vi "Main.vi"(11 "Module Admin":refnum<class "Delacor_lib_QMH_Module Admin.lvclass">) -> ()   [LabVIEW 2026, in "My Singleton Module.lvlib"]
doc: "This template is based off of the Queued Message Handler design pattern and the Queued Message Handler project template that ships with LabVIEW.\n\nThe main difference is that the queue is private to this module and communication between modules is performed via Broadcast and Request events.\n\nRequest events are wrapped in public API methods and are handled in the Event Handling Loop (EHL) of this VI. Any module can register for Broadcast events sent by this module. The EHL generates messages based on user interface actions.\n\nThe Message Handling Loop (MHL) processes messages generated by the EHL, or by other messages. The messages are string values, so new messages can be added easily to the Message Cases case structure in the MHL. Each message cluster can also provide an optional value for Message Data, which is a variant that can be converted to whatever message-specific data is required.\n_____\nBased on DQMH Dev Tools: Project Template 7.1.2.1547."
uses:
  My Singleton Module.lvlib
  <vilib>/Delacor/Delacor QMH/Libraries/Module Admin_class/Delacor_lib_QMH_Module Admin.lvclass
  Module Data--cluster.ctl
  Do Something Argument--cluster.ctl
  <vilib>/Delacor/Delacor QMH/Libraries/Message Queue_class/Delacor_lib_QMH_Message Queue.lvclass/Delacor_lib_QMH_Message Queue.ctl
  Do Something Else Argument--cluster.ctl
  Do Something Else and Wait for Reply Argument--cluster.ctl
  Do Something Else and Wait (Reply Payload)--cluster.ctl
  Stop Argument--cluster.ctl
  <vilib>/Delacor/Delacor QMH/Libraries/Module Admin_class/Delacor_lib_QMH_Module Admin.lvclass/Delacor_lib_QMH_Module Admin.ctl
  Suma 2 Numeros Argument--cluster.ctl
  Suma 2 Numeros (Reply Payload)--cluster.ctl
  Crear Canales DAQ Argument--cluster.ctl
  Start Acquisition Argument--cluster.ctl
  Acquire Argument--cluster.ctl
  Acquire (Reply Payload)--cluster.ctl
  Stop Acquiring Argument--cluster.ctl
  <vilib>/Utility/miscctls.llb/LVPointTypeDef.ctl
  <vilib>/Delacor/Delacor QMH/Libraries/Message Queue_class/Delacor_lib_QMH_Enqueue Message (Single).vi
  <vilib>/Delacor/Delacor QMH/Libraries/Module Admin_class/Delacor_lib_QMH_Get External Launch.vi
  <vilib>/DAQmx/read.llb/DAQmx Read (Analog 1D Wfm NChan NSamp).vi
  <vilib>/DAQmx/miscellaneous.llb/DAQmx Fill In Error Info.vi
  <vilib>/Delacor/Delacor QMH/Libraries/Message Queue_class/Delacor_lib_QMH_Message Queue.lvclass
  DAQ/DAQ.lvlib
panel:
  out "error out":errorcluster
  out "X":dbl
  out "Status":string
  in  "Simulate MHL Error":bool
  in  "Simulate EHL Error":bool
  in  "Do Something Else <Replace Me>":bool
  in  "Do Something <Replace Me>":bool
  # "These controls have associated \"Value Changed\" events configured in the Event Structure on the diagram.\n\nReplace them (and reconfigure the Event Structure) with the controls you need for your application. \n\nOther processes communicate with this Module via its Public API (wrappers for its Request Events).\n\nThis Module communicates with other processes via its Broadcast Events.\nAny process that wants to receive these messages can register for this module's Broadcast events."
  # "This template is for the DQMH framework. See the block diagram for more information on how to use this template."
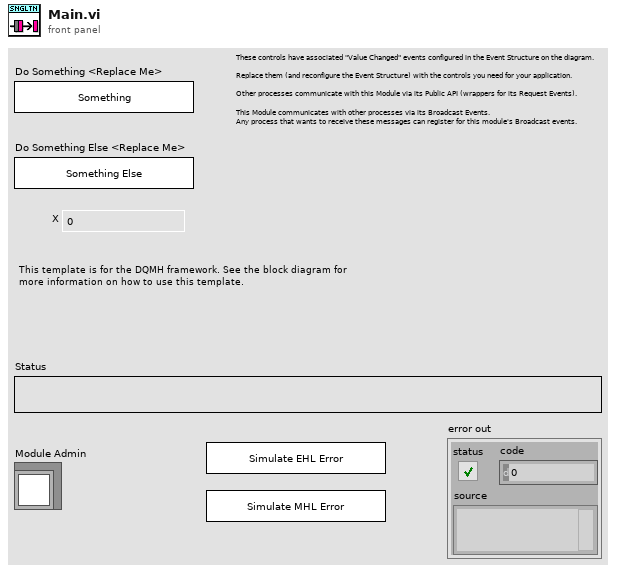
[diagram p1: front panel]
types:
  T1 = typedef "My Singleton Module.lvlib/Request Events--cluster.ctl" = cluster{"Stop Module":refnum<user-event>, "Do Something":refnum<user-event>, "Do Something Else":refnum<user-event>, "Do Something Else and Wait for Reply":refnum<user-event>, "Show Panel":refnum<user-event>, "Hide Panel":refnum<user-event>, "Get Module Execution Status":refnum<user-event>, "Show Diagram":refnum<user-event>, "Suma 2 Numeros":refnum<user-event>, "Crear Canales DAQ":refnum<user-event>, "Start Acquisition":refnum<user-event>, "Acquire":refnum<user-event>, "Stop Acquiring":refnum<user-event>}
  T2 = typedef "My Singleton Module.lvlib/Module Data--cluster.ctl" = cluster{"Status":string, "task out":refnum<k21>}
  T3 = typedef "My Singleton Module.lvlib/Do Something Argument--cluster.ctl" = cluster{"Do Something Msg":string}
  T4 = typedef "My Singleton Module.lvlib/Do Something Else Argument--cluster.ctl" = cluster{"Do Something Else Msg":string, "X":dbl}
  T5 = typedef "My Singleton Module.lvlib/Do Something Else and Wait for Reply Argument--cluster.ctl" = cluster{"Do Something Else Msg":string, "X":dbl, "Wait Notifier":refnum<notifier>, "wait for reply":bool}
  T6 = enum32{"invalid lock state", "Not Locked", "Locked (No Password)", "Password-protected"}
  T7 = typedef "My Singleton Module.lvlib/Stop Argument--cluster.ctl" = cluster{"Origin":string, "Exit via Stop Module Req?":bool, "Wait for Module to stop?":bool}
  T8 = typedef "My Singleton Module.lvlib/Suma 2 Numeros Argument--cluster.ctl" = cluster{"A":dbl, "B":dbl, "Wait Notifier":refnum<notifier>, "wait for reply":bool}
  T9 = typedef "My Singleton Module.lvlib/Crear Canales DAQ Argument--cluster.ctl" = cluster{"Boolean":bool}
  T10 = typedef "My Singleton Module.lvlib/Start Acquisition Argument--cluster.ctl" = cluster{"Boolean":bool}
  T11 = typedef "My Singleton Module.lvlib/Acquire Argument--cluster.ctl" = cluster{"Wait Notifier":refnum<notifier>, "wait for reply":bool}
  T12 = typedef "My Singleton Module.lvlib/Stop Acquiring Argument--cluster.ctl" = cluster{"Boolean":bool}
  T13 = typedef "LVPointTypeDef.ctl" = cluster{"Horizontal":i16, "Vertical":i16}
  T14 = enum32{"Invalid", "Standard", "Closed", "Hidden", "Minimized", "Maximized"}
  T15 = typedef "My Singleton Module.lvlib/Do Something Else and Wait (Reply Payload)--cluster.ctl" = cluster{"Value":dbl, "error":errorcluster}
  T16 = typedef "My Singleton Module.lvlib/Suma 2 Numeros (Reply Payload)--cluster.ctl" = cluster{"A+B":dbl, "error":errorcluster}
  T17 = typedef "My Singleton Module.lvlib/Acquire (Reply Payload)--cluster.ctl" = cluster{"data":waveform(dbl)[], "error":errorcluster}
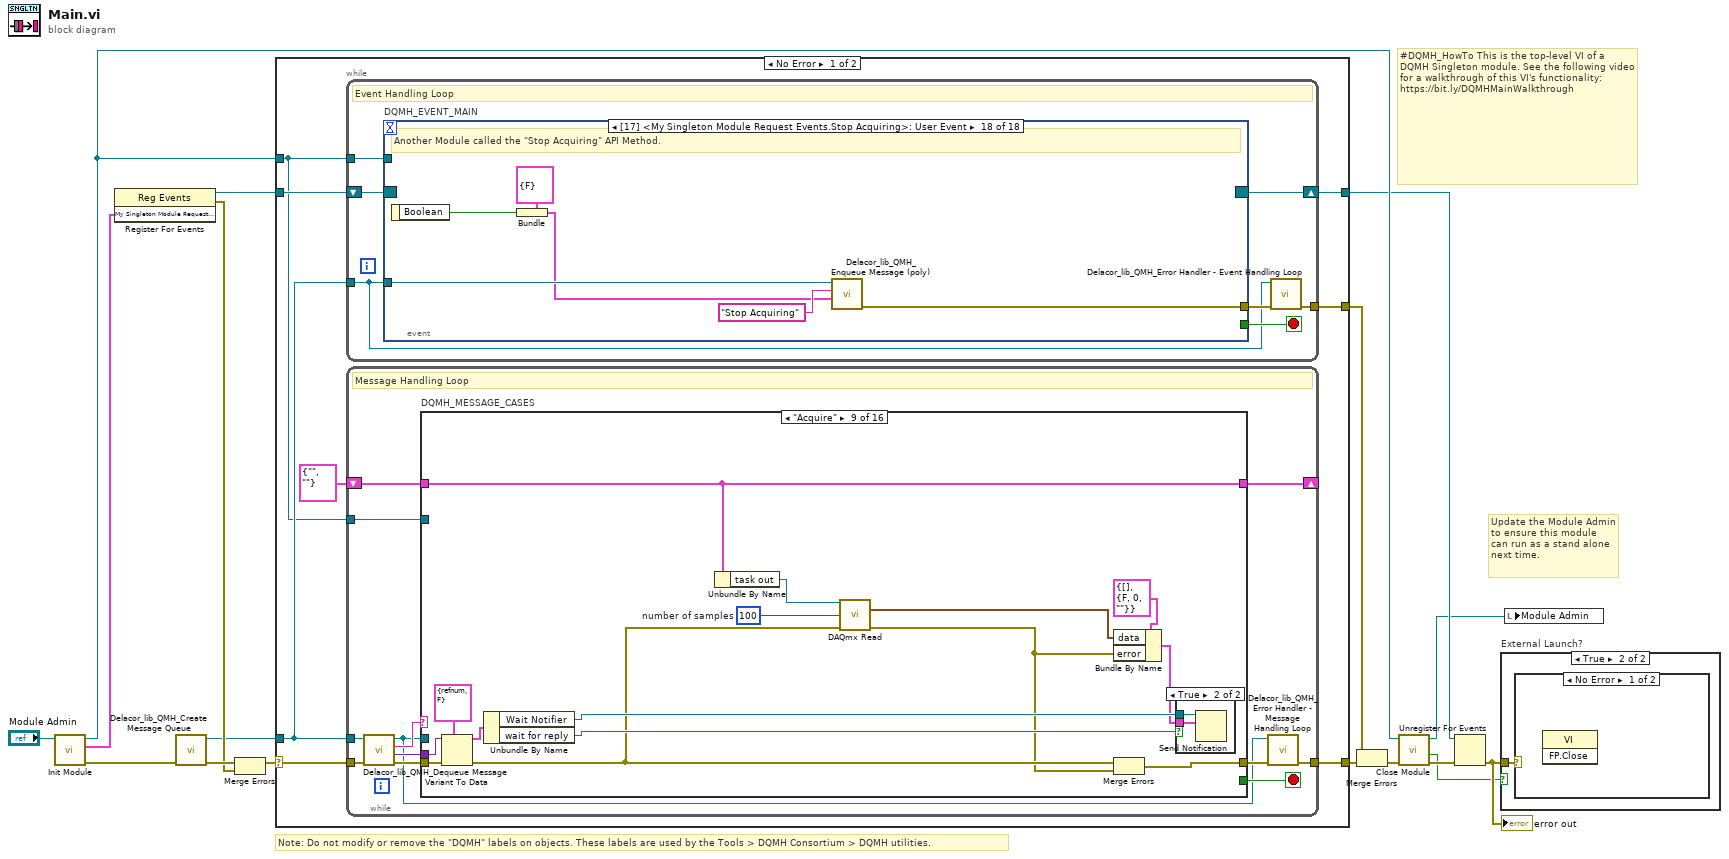
[diagram p0: block diagram]
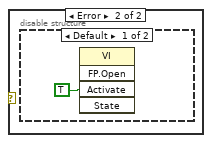
[diagram p3: hidden frame]
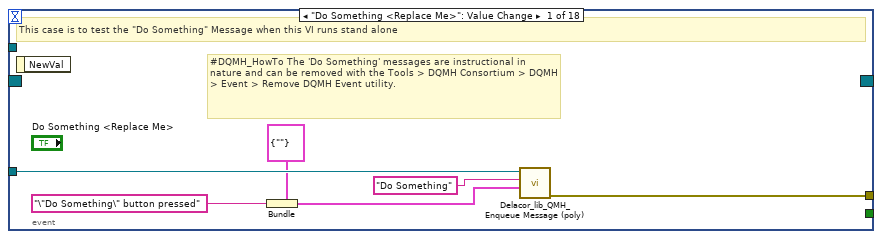
[diagram p5: hidden frame]
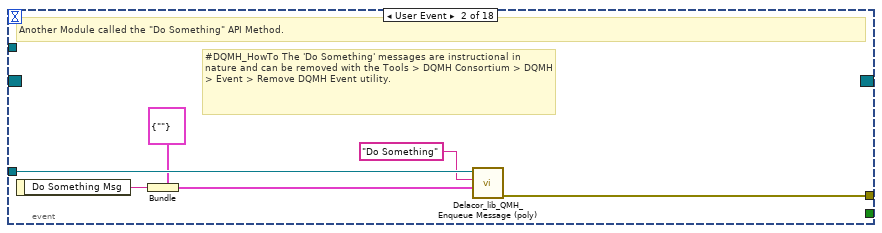
[diagram p6: hidden frame]
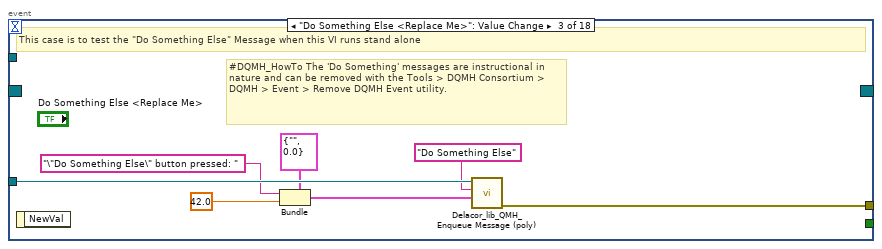
[diagram p7: hidden frame]
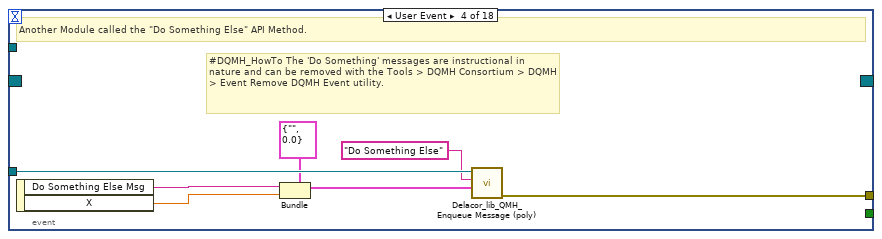
[diagram p8: hidden frame]
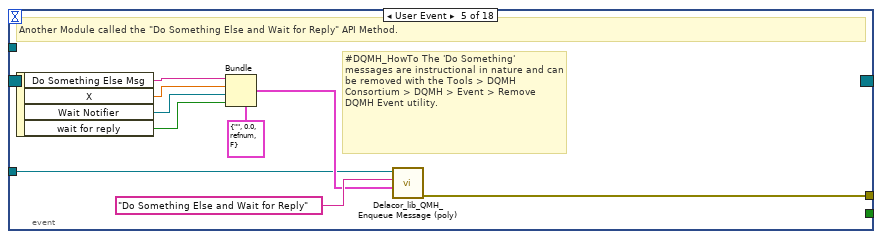
[diagram p9: hidden frame]
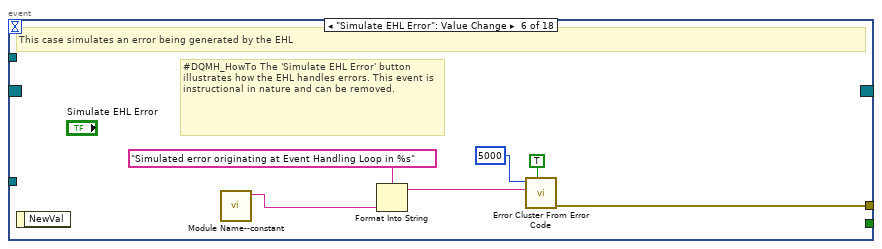
[diagram p10: hidden frame]
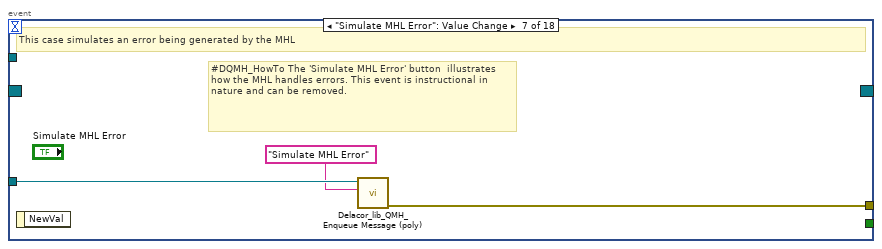
[diagram p11: hidden frame]
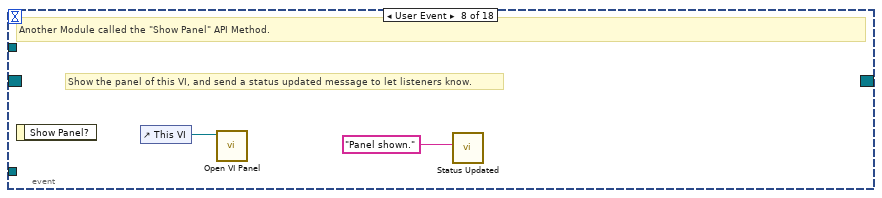
[diagram p12: hidden frame]
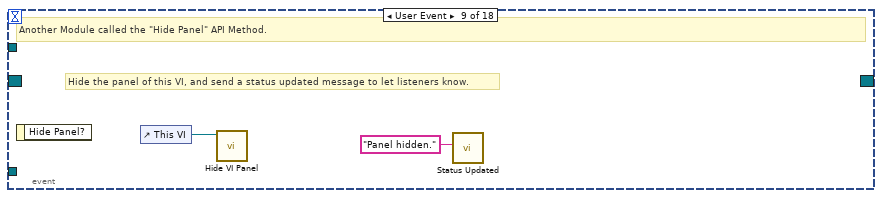
[diagram p13: hidden frame]
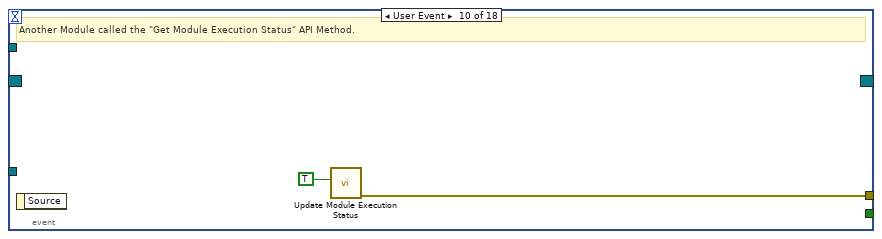
[diagram p14: hidden frame]
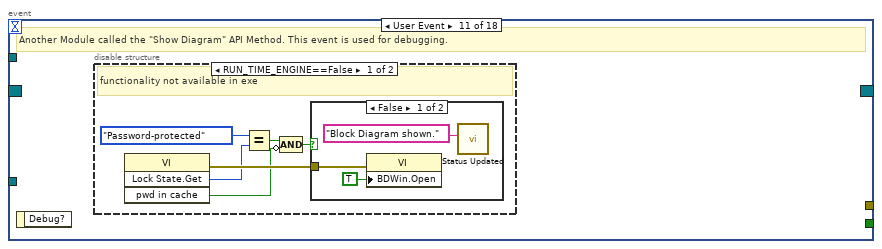
[diagram p15: hidden frame]
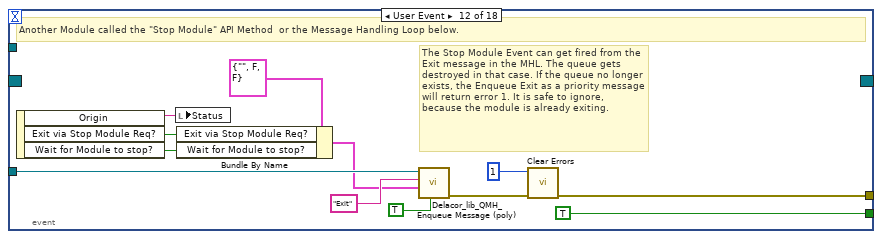
[diagram p18: hidden frame]
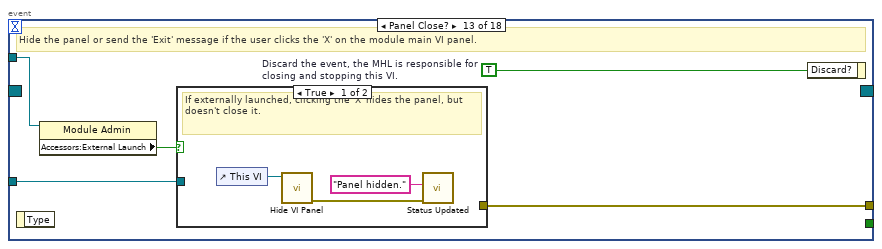
[diagram p19: hidden frame]
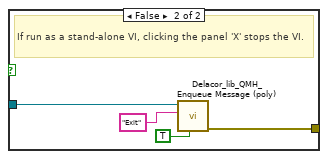
[diagram p20: hidden frame]
diagram:
  # "#DQMH_HowTo This is the top-level VI of a DQMH Singleton module. See the following video for a walkthrough of this VI's functionality: https://bit.ly/DQMHMainWalkthrough"
  # "Note: Do not modify or remove the \"DQMH\" labels on objects. These labels are used by the Tools > DQMH Consortium > DQMH utilities."
  # "Update the Module Admin to ensure this module can run as a stand alone next time."
  n1 = call "Init Module.vi"("Singleton Module Admin in"="Module Admin") -> ("error out"=w16:errorcluster, "My Singleton Module Request Events"=w5:T1, "Singleton Module Admin out"=w8:refnum<class "Delacor_lib_QMH_Module Admin.lvclass">)  [unwired: 8 in]
  n2 = register-events ("DQMH_REG_EVENTS")(w5) -> (reference out=w6:refnum<event-registration>, error out=w9:errorcluster)  [unwired: 2 in]
  n3 = call <vilib>:"Delacor_lib_QMH_Create Message Queue.vi"("error in"=w16) -> ("error out"=w11:errorcluster, "Message Queue"=w4:refnum<class "Delacor_lib_QMH_Message Queue.lvclass">)  [unwired: 9 in]
  n4 = Merge Errors(w11, w9) -> (w10:errorcluster)
  n5 = case shown="No Error" w10 {
    selector: w10 -> [w23 w357]
    tunnel: [w25 w356] -> w17
    tunnel: [w22 w355] -> w7
    tunnel: w6 -> [w20 w355]
    tunnel: w4 -> [w19 w350]
    tunnel: [w24 _] -> w14
    tunnel: w8 -> [w18 w351]
    frame No Error {
      n6 = while {
        tunnel: w19 -> [w26]
        shift-right: [w29] -> w22
        shift-left: w20 -> [w30]
        tunnel: [w31] -> w24
        tunnel: w18 -> [w27]
        stop <- w28 stop-if-true
        # "Event Handling Loop"
        n7 = event "DQMH_EVENT_MAIN" shown="[17] <My Singleton Module Request Events.Stop Acquiring>: User Event" {
          selector: w30 -> [_ _ _ _ _ _ _ _ _ _ _ _ _ _ _ _ _ _]
          dyn-events: [_ _ _ _ _ _ _ _ _ _ _ _ _ _ _ _ _ _] -> w29
          timeout: _ -> [_ _ _ _ _ _ _ _ _ _ _ _ _ _ _ _ _ _]
          tunnel: [_ _ _ _ _ _ _ _ _ _ _ TRUE ("Discard?") _ _ _ _ _ _] -> w28
          tunnel: w26 -> [w37 w43 w50 w57 w60 _ w75 _ _ _ _ w99 w106 w124 w130 w136 w143 w149]
          tunnel: [w38 w44 w51 w58 w67 w73 w76 _ _ w82 _ w102 w108 w116 w125 w133 w137 w144] -> w32
          tunnel: w27 -> [_ _ _ _ _ _ _ _ _ _ _ _ w105 _ _ _ _ _]
          event "Do Something <Replace Me>": Value Change {
            # "#DQMH_HowTo The 'Do Something' messages are instructional in nature and can be removed with the Tools > DQMH Consortium > DQMH > Event > Remove DQMH Event utility."
            # "This case is to test the \"Do Something\" Message when this VI runs stand alone"
            n8 = event-data() -> ()  [unwired: 1 in, 1 out]
            n9 = Bundle(cluster=T3 {"Do Something Msg"=""} ("Do Something Argument"), "Do Something Msg"="\"Do Something\" button pressed" ("\"Do Something\" button pressed")) -> (w33:T3)
            n10 = call-poly <vilib>:"Delacor_lib_QMH_Enqueue Message (poly).vi"("Message Data"=w33, "Message"="Do Something", "Message Queue in"=w37) -> ("error out"=w38:errorcluster)  [unwired: 7 in, 1 out]
          }
          event User Event {
            # "#DQMH_HowTo The 'Do Something' messages are instructional in nature and can be removed with the Tools > DQMH Consortium > DQMH > Event > Remove DQMH Event utility."
            # "Another Module called the \"Do Something\" API Method."
            n11 = event-data() -> ("Do Something Msg"=w40:string)  [unwired: 1 in]
            n12 = Bundle(cluster=T3 {"Do Something Msg"=""} ("Do Something Argument"), "Do Something Msg"=w40) -> (w39:T3)
            n13 = call-poly <vilib>:"Delacor_lib_QMH_Enqueue Message (poly).vi"("Message Data"=w39, "Message"="Do Something", "Message Queue in"=w43) -> ("error out"=w44:errorcluster)  [unwired: 7 in, 1 out]
          }
          event "Do Something Else <Replace Me>": Value Change {
            # "#DQMH_HowTo The 'Do Something' messages are instructional in nature and can be removed with the Tools > DQMH Consortium > DQMH > Event > Remove DQMH Event utility."
            # "This case is to test the \"Do Something Else\" Message when this VI runs stand alone"
            n14 = event-data() -> ()  [unwired: 1 in, 1 out]
            n15 = Bundle(cluster=T4 {"Do Something Else Msg"="", "X"=0.0} ("Do Something Else Argument"), "Do Something Else Msg"="\"Do Something Else\" button pressed: " ("\"Do Something Else\" button pressed"), "X"=42.0) -> (w47:T4)
            n16 = call-poly <vilib>:"Delacor_lib_QMH_Enqueue Message (poly).vi"("Message Data"=w47, "Message"="Do Something Else", "Message Queue in"=w50) -> ("error out"=w51:errorcluster)  [unwired: 7 in, 1 out]
          }
          event User Event {
            # "#DQMH_HowTo The 'Do Something' messages are instructional in nature and can be removed with the Tools > DQMH Consortium > DQMH > Event Remove DQMH Event utility."
            # "Another Module called the \"Do Something Else\" API Method."
            n17 = event-data() -> ("Do Something Else Msg"=w53:string, "X"=w52:dbl)  [unwired: 1 in]
            n18 = Bundle(cluster=T4 {"Do Something Else Msg"="", "X"=0.0} ("Do Something Else Argument"), "Do Something Else Msg"=w53, "X"=w52) -> (w54:T4)
            n19 = call-poly <vilib>:"Delacor_lib_QMH_Enqueue Message (poly).vi"("Message Data"=w54, "Message"="Do Something Else", "Message Queue in"=w57) -> ("error out"=w58:errorcluster)  [unwired: 7 in, 1 out]
          }
          event User Event {
            # "#DQMH_HowTo The 'Do Something' messages are instructional in nature and can be removed with the Tools > DQMH Consortium > DQMH > Event > Remove DQMH Event utility."
            # "Another Module called the \"Do Something Else and Wait for Reply\" API Method."
            n20 = event-data() -> ("Do Something Else Msg"=w63:string, "X"=w62:dbl, "Wait Notifier"=w61:refnum<notifier>, "wait for reply"=w59:bool)  [unwired: 1 in]
            n21 = Bundle(cluster=T5 {"Do Something Else Msg"="", "X"=0.0, "Wait Notifier"=refnum, "wait for reply"=FALSE} ("Do Something Else and Wait for Reply Argument"), "Do Something Else Msg"=w63, "X"=w62, "Wait Notifier"=w61, "wait for reply"=w59) -> (w64:T5)
            n22 = call-poly <vilib>:"Delacor_lib_QMH_Enqueue Message (poly).vi"("Message Data"=w64, "Message"="Do Something Else and Wait for Reply", "Message Queue in"=w60) -> ("error out"=w67:errorcluster)  [unwired: 7 in, 1 out]
          }
          event "Simulate EHL Error": Value Change {
            # "#DQMH_HowTo The 'Simulate EHL Error' button  illustrates how the EHL handles errors. This event is instructional in nature and can be removed."
            # "This case simulates an error being generated by the EHL"
            n23 = event-data() -> ()  [unwired: 1 in, 1 out]
            n24 = call "Module Name--constant.vi"() -> ("Module Name"=w70:string)  [unwired: 11 in]
            n25 = Format Into String(format string="Simulated error originating at Event Handling Loop in %s", w70) -> (resulting string=w71:string)  [unwired: 2 in, 1 out]
            n26 = call <vilib>:"Error Cluster From Error Code.vi"("show call chain? (False)"=TRUE, "error message (\"\")"=w71, "error code (0)"=5000) -> ("error out"=w73:errorcluster)  [unwired: 6 in]
          }
          event "Simulate MHL Error": Value Change {
            # "#DQMH_HowTo The 'Simulate MHL Error' button  illustrates how the MHL handles errors. This event is instructional in nature and can be removed."
            # "This case simulates an error being generated by the MHL"
            n27 = event-data() -> ()  [unwired: 1 in, 1 out]
            n28 = call-poly <vilib>:"Delacor_lib_QMH_Enqueue Message (poly).vi"("Message"="Simulate MHL Error", "Message Queue in"=w75) -> ("error out"=w76:errorcluster)  [unwired: 8 in, 1 out]
          }
          event User Event {
            # "Show the panel of this VI, and send a status updated message to let listeners know."
            # "Another Module called the \"Show Panel\" API Method."
            n29 = event-data() -> ()  [unwired: 1 in, 1 out]
            n30 = control-ref of="This VI"() -> (w78:refnum<vi>)
            n31 = call "Open VI Panel.vi"("VI"=w78) -> ()  [unwired: 10 in, 1 out]
            n32 = call "Status Updated.vi"("Status"="Panel shown." ("format string")) -> ()  [unwired: 10 in, 1 out]
          }
          event User Event {
            # "Hide the panel of this VI, and send a status updated message to let listeners know."
            # "Another Module called the \"Hide Panel\" API Method."
            n33 = event-data() -> ()  [unwired: 1 in, 1 out]
            n34 = control-ref of="This VI"() -> (w80:refnum<vi>)
            n35 = call "Hide VI Panel.vi"("VI"=w80) -> ()  [unwired: 10 in, 1 out]
            n36 = call "Status Updated.vi"("Status"="Panel hidden." ("format string")) -> ()  [unwired: 10 in, 1 out]
          }
          event User Event {
            # "Another Module called the \"Get Module Execution Status\" API Method."
            n37 = event-data() -> ()  [unwired: 1 in, 1 out]
            n38 = call "Update Module Execution Status.vi"("Running?"=TRUE) -> ("error out"=w82:errorcluster)  [unwired: 10 in]
          }
          event User Event {
            # "Another Module called the \"Show Diagram\" API Method. This event is used for debugging."
            n39 = event-data() -> ()  [unwired: 1 in, 1 out]
            n40 = disable-structure shown="RUN_TIME_ENGINE==False" {
              frame condition #0 (active) {
                # "functionality not available in exe"
                n41 = invoke on="Invoke Node" class="VI" method="Lock State.Get"() -> (error out=w88:errorcluster, "Get Lock State"=w87:T6, "pwd in cache"=w84:bool)  [unwired: 4 in, 1 out]
                n42 = Equal?(x=T6."Password-protected", y=w87) -> (x = y?=w85:bool)
                n43 = Compound Arithmetic op=AND(w85, invert w84) -> (w83:bool)
                n44 = case shown="False" w83 {
                  tunnel: w88 -> [w91 _]
                  frame False {
                    n45 = property on="Property Node" class="VI"(error in=w91, "BDWin.Open"=TRUE ("Block Diagram Window:Open")) -> ()  [unwired: 1 in, 2 out]
                    n46 = call "Status Updated.vi"("Status"="Block Diagram shown." ("format string")) -> ()  [unwired: 10 in, 1 out]
                  }
                  frame True {
                    # "Password-protected VI, and the password is not in the cache. Do not show the diagram."
                  }
                }
              }
              frame condition #1 {
              }
            }
          }
          event User Event {
            # "The Stop Module Event can get fired from the Exit message in the MHL. The queue gets destroyed in that case. If the queue no longer exists, the Enqueue Exit as a priority message will return error 1. It is safe to ignore, because the module is already exiting."
            # "Another Module called the \"Stop Module\" API Method  or the Message Handling Loop below."
            n47 = event-data() -> ("Origin"=w98:string, "Exit via Stop Module Req?"=w94:bool, "Wait for Module to stop?"=w93:bool)  [unwired: 1 in]
            n48 = local write "Status"(w98) -> ()
            n49 = Bundle By Name(cluster=T7 {"Origin"="", "Exit via Stop Module Req?"=FALSE, "Wait for Module to stop?"=FALSE} ("Stop Argument"), "Exit via Stop Module Req?"=w94, "Wait for Module to stop?"=w93) -> (w92:T7)
            n50 = call-poly <vilib>:"Delacor_lib_QMH_Enqueue Message (poly).vi"("Priority Message? (F)"=TRUE, "Message Data"=w92, "Message"="Exit", "Message Queue in"=w99) -> ("error out"=w103:errorcluster)  [unwired: 6 in, 1 out]
            n51 = call <vilib>:"Clear Errors.vi"("error in (no error)"=w103, "specific error code to clear (0: all)"=1) -> ("error out"=w102:errorcluster)  [unwired: 4 in, 1 out]
          }
          event Panel Close? {
            w107 = TRUE  # Discard the event, the MHL is responsible for closing and stopping this VI.
            # "Hide the panel or send the 'Exit' message if the user clicks the 'X' on the module main VI panel."
            n52 = event-data() -> ()  [unwired: 1 in, 1 out]
            n53 = property on="Property Node" class="Module Admin"(reference=w105) -> ("Accessors:External Launch"=w104:bool)  [unwired: 1 in, 2 out]
            n54 = case shown="True" w104 {
              tunnel: w106 -> [_ w114]
              tunnel: [_ w115] -> w108
              frame True {
                # "If externally launched, clicking the 'X' hides the panel, but doesn't close it."
                n55 = control-ref of="This VI"() -> (w111:refnum<vi>)
                n56 = call "Hide VI Panel.vi"("VI"=w111) -> ("error out"=w109:errorcluster)  [unwired: 10 in]
                n57 = call "Status Updated.vi"("error in"=w109, "Status"="Panel hidden." ("format string")) -> ()  [unwired: 9 in, 1 out]
              }
              frame False {
                # "If run as a stand-alone VI, clicking the panel 'X' stops the VI."
                n58 = call-poly <vilib>:"Delacor_lib_QMH_Enqueue Message (poly).vi"("Priority Message? (F)"=TRUE, "Message"="Exit", "Message Queue in"=w114) -> ("error out"=w115:errorcluster)  [unwired: 7 in, 1 out]
              }
            }
            n59 = event-data ("Event Filter Node")("Discard?"=w107) -> ()  [unwired: 1 in, 1 out]
          }
          event User Event {
            # "Another Module called the \"Suma 2 Numeros\" API Method."
            n60 = event-data() -> ("A"=w120:dbl, "B"=w119:dbl, "Wait Notifier"=w118:refnum<notifier>, "wait for reply"=w117:bool)  [unwired: 1 in]
            n61 = Bundle(cluster=T8 {"A"=0.0, "B"=0.0, "Wait Notifier"=refnum, "wait for reply"=FALSE} ("Suma 2 Numeros Argument"), "A"=w120, "B"=w119, "Wait Notifier"=w118, "wait for reply"=w117) -> (w121:T8)
            n62 = call-poly <vilib>:"Delacor_lib_QMH_Enqueue Message (poly).vi"("Message Data"=w121, "Message"="Suma 2 Numeros", "Message Queue in"=w124) -> ("error out"=w116:errorcluster)  [unwired: 7 in, 1 out]
          }
          event User Event {
            # "Another Module called the \"Crear Canales DAQ\" API Method."
            n63 = event-data() -> ("Boolean"=w126:bool)  [unwired: 1 in]
            n64 = Bundle(cluster=T9 {"Boolean"=FALSE} ("Crear Canales DAQ Argument"), "Boolean"=w126) -> (w127:T9)
            n65 = call-poly <vilib>:"Delacor_lib_QMH_Enqueue Message (poly).vi"("Message Data"=w127, "Message"="Crear Canales DAQ", "Message Queue in"=w130) -> ("error out"=w125:errorcluster)  [unwired: 7 in, 1 out]
          }
          event User Event {
            # "Another Module called the \"Start Acquisition\" API Method."
            n66 = event-data() -> ("Boolean"=w131:bool)  [unwired: 1 in]
            n67 = Bundle(cluster=T10 {"Boolean"=FALSE} ("Start Acquisition Argument"), "Boolean"=w131) -> (w132:T10)
            n68 = call-poly <vilib>:"Delacor_lib_QMH_Enqueue Message (poly).vi"("Message Data"=w132, "Message"="Start Acquisition", "Message Queue in"=w136) -> ("error out"=w133:errorcluster)  [unwired: 7 in, 1 out]
          }
          event User Event {
            # "Another Module called the \"Acquire\" API Method."
            n69 = event-data() -> ("Wait Notifier"=w139:refnum<notifier>, "wait for reply"=w138:bool)  [unwired: 1 in]
            n70 = Bundle(cluster=T11 {"Wait Notifier"=refnum, "wait for reply"=FALSE} ("Acquire Argument"), "Wait Notifier"=w139, "wait for reply"=w138) -> (w140:T11)
            n71 = call-poly <vilib>:"Delacor_lib_QMH_Enqueue Message (poly).vi"("Message Data"=w140, "Message"="Acquire", "Message Queue in"=w143) -> ("error out"=w137:errorcluster)  [unwired: 7 in, 1 out]
          }
          event User Event {
            # "Another Module called the \"Stop Acquiring\" API Method."
            n72 = event-data() -> ("Boolean"=w145:bool)  [unwired: 1 in]
            n73 = Bundle(cluster=T12 {"Boolean"=FALSE} ("Stop Acquiring Argument"), "Boolean"=w145) -> (w146:T12)
            n74 = call-poly <vilib>:"Delacor_lib_QMH_Enqueue Message (poly).vi"("Message Data"=w146, "Message"="Stop Acquiring", "Message Queue in"=w149) -> ("error out"=w144:errorcluster)  [unwired: 7 in, 1 out]
          }
        }
        n75 = call-dynamic "Delacor_lib_QMH_Error Handler - Event Handling Loop.vi"("error in"=w32, "Message Queue in"=w26) -> ("dup error in"=w31:errorcluster)  [unwired: 8 in, 1 out]
      }
      n76 = while {
        tunnel: w19 -> [w150]
        shift-right: [w158] -> _
        shift-left: T2 {"Status"="", "task out"=""} ("Data Cluster") -> [w159]
        tunnel: w23 -> [w161]
        tunnel: [w153] -> w25
        tunnel: w18 -> [w154]
        stop <- w157 stop-if-true
        # "Message Handling Loop"
        n77 = call-dynamic "Delacor_lib_QMH_Dequeue Message.vi"("error in"=w161, "Message Queue in"=w150) -> ("error out"=w160:errorcluster, "Message Data"=w155:variant, "Message"=w156:string, "Message Queue out"=w151:refnum<class "Delacor_lib_QMH_Message Queue.lvclass">)  [unwired: 6 in]
        n78 = case "DQMH_MESSAGE_CASES" shown="\"Acquire\"" w156 {
          selector: w156 -> [_ _ _ _ _ _ _ _ _ _ _ _ _ _ _ w345]
          tunnel: w151 -> [_ _ _ _ _ _ _ _ _ _ _ _ _ w311 w333 _]
          tunnel: w160 -> [w179 w183 w191 w200 w219 w245 w256 w264 w283 w293 w296 w298 w307 w318 w339 w348]
          tunnel: [w177 w183 w189 w199 w218 w235 w250 w259 w275 w288 w295 w298 w306 w314 w334 w349] -> w152
          tunnel: w159 -> [w168 w182 w188 w198 w215 w244 w255 w258 w271 w287 w294 w297 w304 w313 w332 w346]
          tunnel: [w167 w182 w188 w198 w215 w244 w249 w257 w271 w287 w294 w297 w304 w313 w332 w346] -> w158
          tunnel: [_ _ _ _ _ _ _ _ _ _ _ _ _ _ w331 _] -> w157
          tunnel: w155 -> [_ _ w187 w195 w212 w242 w254 w263 w282 w291 _ _ _ w312 w330 _]
          tunnel: w154 -> [w169 _ _ _ _ _ _ _ _ _ _ _ _ w310 w325 _]
          frame "Initialize" {
            w163 = "Initial Message" ("Initial Message")
            # "#DQMH_CodeNeeded - Initialize the appearance of the front panel."
            # "#DQMH_CodeNeeded - Initialize your state data here."
            # "Initialize - Any operation that needs to be done before the module can receive messages. Synchronize Caller Events.vi will inform Start Module.vi that the module has launched and is ready to receive messages. Module Did Init.vi will broadcast that the module initialized."
            n79 = call "Synchronize Caller Events.vi"("error in"=w179, "Singleton Module Admin in"=w169) -> ("error out"=w178:errorcluster, "Singleton Module Admin out"=w164:refnum<class "Delacor_lib_QMH_Module Admin.lvclass">)  [unwired: 8 in]
            n80 = property on="Property Node" class="Module Admin"(reference=w164) -> ("Accessors:External Launch"=w173:bool)  [unwired: 1 in, 2 out]
            n81 = Select(t=T14."Hidden" ("State"), s=w173, f=T14."Standard" ("State")) -> (s? t:f=w170:T14)
            n82 = call "Module Name--constant.vi"() -> ("Module Name"=w176:string)  [unwired: 11 in]
            n83 = property on="Property Node" class="VI"("Front Panel.Title"=w176) -> (reference out=w175:refnum<vi>, error out=w181:errorcluster)  [unwired: 2 in]
            n84 = invoke on="Invoke Node" class="VI" method="FP.Open"(reference=w175, error in=w181, "State"=w170) -> (reference out=w174:refnum<vi>, error out=w180:errorcluster)  [unwired: 2 in, 3 out]
            n85 = Bundle By Name(cluster=w168, "Status"=w163) -> (w167:T2)
            n86 = invoke on="Invoke Node" class="VI" method="FP.Center"(reference=w174, error in=w180) -> ()  [unwired: 1 in, 3 out]
            n87 = property on="Pane" class="Pane"("Origin"=T13 {"Horizontal"=0, "Vertical"=0}) -> ()  [unwired: 2 in, 2 out]
            n88 = call "Module Name--constant.vi"() -> ("Module Name"=w165:string)  [unwired: 11 in]
            n89 = call "Module Did Init.vi"("error in"=w178, "Initialized?"=TRUE, "Origin"=w165) -> ("error out"=w177:errorcluster)  [unwired: 8 in]
            "Status" <- w163
          }
          frame "---Module Specific---" {
            # "Separator -- The following cases handle messages specific to this Module."
          }
          frame "Do Something" {
            # "#DQMH_HowTo The 'Do Something' messages are instructional in nature and can be removed with the Tools > DQMH Consortium > DQMH > Event > Remove DQMH Event utility."
            # "Do Something - Replace this message with functionality for your own application. Note that this message also fires the \"Did Something\" broadcast event."
            n90 = Variant To Data(error in=w191, type=T3 {"Do Something Msg"=""} ("Do Something Argument"), Variant=w187) -> (data=w186:T3, error out=w190:errorcluster)
            n91 = Unbundle By Name(w186) -> ("Do Something Msg"=w184:string)
            n92 = call "Did Something.vi"("error in"=w190, "Did Something Msg"=w184) -> ("error out"=w189:errorcluster)  [unwired: 9 in]
            n93 = local write "Status"(w184) -> ()
            n94 = call "Status Updated.vi"("Status"=w184) -> ()  [unwired: 10 in, 1 out]
          }
          frame "Do Something Else" {
            # "#DQMH_HowTo The 'Do Something' messages are instructional in nature and can be removed with the Tools > DQMH Consortium > DQMH > Event > Remove DQMH Event utility."
            # "Do Something Else - Replace this message with functionality for your own application."
            n95 = Variant To Data(error in=w200, type=T4 {"Do Something Else Msg"="", "X"=0.0} ("Do Something Else Argument"), Variant=w195) -> (data=w196:T4, error out=w199:errorcluster)
            n96 = Unbundle By Name(w196) -> ("Do Something Else Msg"=w194:string, "X"=w193:dbl)
            "X" <- w193
            n97 = Format Into String(initial string=w194, w193) -> (resulting string=w192:string)  [unwired: 2 in, 1 out]
            n98 = local write "Status"(w192) -> ()
            n99 = call "Status Updated.vi"("Status"=w192) -> ()  [unwired: 10 in, 1 out]
          }
          frame "Do Something Else and Wait for Reply" {
            w207 = "X(%.2f)+Offset(%.2f)=%.2f"  # status message format string
            # "#DQMH_HowTo The 'Do Something' messages are instructional in nature and can be removed."
            # "Send back X with a random offset"
            # "Do Something Else and Wait for Reply - Replace this message with functionality for your own application. Note that this message must fire a notifier to let callers know it has finished execution, and it returns an error if the 'Value' is negative."
            n100 = Variant To Data(error in=w219, type=T5 {"Do Something Else Msg"="", "X"=0.0, "Wait Notifier"=refnum, "wait for reply"=FALSE} ("Do Something Else and Wait for Reply Argument"), Variant=w212) -> (data=w213:T5, error out=w217:errorcluster)
            n101 = Unbundle By Name(w213) -> ("Wait Notifier"=w201:refnum<notifier>, "Do Something Else Msg"=w211:string, "X"=w208:dbl, "wait for reply"=w204:bool)
            n102 = Random Number (0-1)() -> (number: 0 to 1=w209:dbl)
            n103 = Add(x=w209, y=w208) -> (x+y=w203:dbl)
            n104 = Less Than 0?(x=w203) -> (x < 0?=w206:bool)
            n105 = local write "X"(w208) -> ()
            n106 = case shown="True" w206 {
              tunnel: [_ w229] -> w216
              frame False {
              }
              frame True {
                n107 = call <vilib>:"Error Cluster From Error Code.vi"("show call chain? (False)"=TRUE, "error message (\"\")"="The 'Something Else and Wait for Reply' message generated a negative number, which is considered an error condition.", "error code (0)"=5000) -> ("error out"=w229:errorcluster)  [unwired: 6 in]
              }
            }
            n108 = Format Into String(format string=w207, initial string=w211, w208, w209, w203) -> (resulting string=w205:string)  [unwired: 1 in, 1 out]
            n109 = Bundle By Name(cluster=T15 {"Value"=0.0, "error"={"status"=FALSE, "code"=0, "source"=""}} ("notification"), "error"=w216, "Value"=w203) -> (w202:T15)
            n110 = local write "Status"(w205) -> ()
            n111 = call "Status Updated.vi"("Status"=w205) -> ()  [unwired: 10 in, 1 out]
            n112 = case shown="True" w204 {
              tunnel: w202 -> [_ w222]
              tunnel: w201 -> [_ w221]
              frame False {
              }
              frame True {
                # "Simulate an operation that requires a wait."
                n113 = flat-sequence {
                  tunnel: w222 -> [w225]
                  tunnel: w221 -> [w224]
                  tunnel: w220 -> [_]
                  frame #0 {
                    n114 = Send Notification(notification=w225, notifier=w224) -> ()  [unwired: 1 in, 2 out]
                  }
                }
                n115 = Wait (ms)(milliseconds to wait=u32 1000) -> (millisecond timer value=w220:u32)
              }
            }
            n116 = Merge Errors(w217, w216) -> (w218:errorcluster)
          }
          frame "Suma 2 Numeros" {
            # "Evento para que el modulo sume 2 numeros"
            n117 = Variant To Data(error in=w245, type=T8 {"A"=0.0, "B"=0.0, "Wait Notifier"=refnum, "wait for reply"=FALSE} ("Suma 2 Numeros Argument"), Variant=w242) -> (data=w240:T8, error out=w243:errorcluster)
            n118 = Unbundle By Name(w240) -> ("A"=w233:dbl, "B"=w232:dbl, "Wait Notifier"=w239:refnum<notifier>, "wait for reply"=w238:bool)
            n119 = Add(x=w233, y=w232) -> (x+y=w230:dbl)
            n120 = Format Into String(format string="a:%.2f,b:%.2f/t a+b:%.2f", w233, w232, w230) -> (resulting string=w234:string)  [unwired: 2 in, 1 out]
            n121 = call "Status Updated.vi"("Status"=w234) -> ()  [unwired: 10 in, 1 out]
            n122 = call "Nuevo resultado de la Suma Actualizado.vi"("A+B"=w230) -> ()  [unwired: 10 in, 1 out]
            n123 = Merge Errors(w243) -> (w235:errorcluster)
            n124 = Bundle By Name(cluster=T16 {"A+B"=0.0, "error"={"status"=FALSE, "code"=0, "source"=""}} ("Suma 2 Numeros (Reply Payload)"), "A+B"=w230) -> (w237:T16)
            n125 = case "DQMH_FIRE_NOTIFIER" shown="True" w238 {
              tunnel: w239 -> [_ w247]
              tunnel: w237 -> [_ w246]
              frame False {
              }
              frame True {
                n126 = Send Notification(notification=w246, notifier=w247) -> ()  [unwired: 1 in, 2 out]
              }
            }
          }
          frame "Crear Canales DAQ" {
            # "Crear Canales DAQmx"
            n127 = Variant To Data(error in=w256, type=T9 {"Boolean"=FALSE} ("Crear Canales DAQ Argument"), Variant=w254) -> (data=w252:T9, error out=w251:errorcluster)
            n128 = Unbundle By Name(w252) -> ()  [unwired: 1 out]
            n129 = call "Crear Canales DAQ.vi"("error in"=w251) -> ("error out"=w250:errorcluster, "task out"=w248:refnum<k21>)  [unwired: 9 in]
            n130 = Bundle By Name(cluster=w255, "task out"=w248) -> (w249:T2)
          }
          frame "Start Acquisition" {
            n131 = Variant To Data(error in=w264, type=T10 {"Boolean"=FALSE} ("Start Acquisition Argument"), Variant=w263) -> (data=w261:T10, error out=w260:errorcluster)
            n132 = Unbundle By Name(w261) -> ()  [unwired: 1 out]
            n133 = in-place {
              in-place-border: w260 -> [w268]
              in-place-border: [w267] -> w259
              n134 = in-place-cluster #1(w258) -> ("task out"=w266:refnum<k21>)
              n135 = call <vilib>:"DAQmx Start Task.vi"("task/channels in"=w266, "error in"=w268) -> ("task out"=w265:refnum<k21>, "error out"=w267:errorcluster)  [unwired: 12 in]
              n136 = in-place-cluster #1("task out"=w265) -> (w257:T2)
            }
          }
          frame "Acquire" {
            w269 = 100  # number of samples
            n137 = Variant To Data(error in=w283, type=T11 {"Wait Notifier"=refnum, "wait for reply"=FALSE} ("Acquire Argument"), Variant=w282) -> (data=w280:T11, error out=w274:errorcluster)
            n138 = Unbundle By Name(w280) -> ("Wait Notifier"=w279:refnum<notifier>, "wait for reply"=w278:bool)
            n139 = Unbundle By Name(w271) -> ("task out"=w270:refnum<k21>)
            n140 = call-poly <vilib>:"DAQmx Read.vi"("task/channels in"=w270, "number of samples per channel"=w269, "error in"=w274) -> ("data"=w272:waveform(dbl)[], "error out"=w273:errorcluster)  [unwired: 10 in, 1 out]
            n141 = Bundle By Name(cluster=T17 {"data"=[], "error"={"status"=FALSE, "code"=0, "source"=""}} ("Acquire (Reply Payload)"), "data"=w272, "error"=w273) -> (w277:T17)
            n142 = Merge Errors(w274, w273) -> (w275:errorcluster)
            n143 = case "DQMH_FIRE_NOTIFIER" shown="True" w278 {
              tunnel: w279 -> [_ w285]
              tunnel: w277 -> [_ w284]
              frame False {
              }
              frame True {
                n144 = Send Notification(notification=w284, notifier=w285) -> ()  [unwired: 1 in, 2 out]
              }
            }
          }
          frame "Stop Acquiring" {
            n145 = Variant To Data(error in=w293, type=T12 {"Boolean"=FALSE} ("Stop Acquiring Argument"), Variant=w291) -> (data=w289:T12, error out=w292:errorcluster)
            n146 = Unbundle By Name(w289) -> ()  [unwired: 1 out]
            n147 = Unbundle By Name(w287) -> ("task out"=w286:refnum<k21>)
            n148 = call <vilib>:"DAQmx Clear Task.vi"("task in"=w286, "error in"=w292) -> ("error out"=w288:errorcluster)  [unwired: 13 in]
          }
          frame "---Copy This Frame---" {
            # "Duplicate this frame when creating new messages.  Change this comment in the duplicated frame to describe this message."
            n149 = Merge Errors(w296) -> (w295:errorcluster)
          }
          frame "---Exit and Error Handling---" {
            # "Separator - The following cases handle errors and exit messages."
          }
          frame "Simulate MHL Error" {
            # "#DQMH_HowTo The 'Simulate MHL Error' button  illustrates how the MHL handles errors. This event is instructional in nature and can be removed."
            # "Simulate an error occurring at the MHL"
            n150 = call "Module Name--constant.vi"() -> ("Module Name"=w300:string)  [unwired: 11 in]
            n151 = Format Into String(format string="Simulated error originating at Message Handling Loop in %s", w300) -> (resulting string=w301:string)  [unwired: 2 in, 1 out]
            n152 = call <vilib>:"Error Cluster From Error Code.vi"("show call chain? (False)"=TRUE, "error message (\"\")"=w301, "error code (0)"=5001) -> ("error out"=w305:errorcluster)  [unwired: 6 in]
            n153 = Merge Errors(w307, w305) -> (w306:errorcluster)
          }
          frame "Error" {
            # "#DQMH_CodeRecommended - If the module is running in standalone mode (External Launch = FALSE), this code will pop up an error dialog and call the 'Exit' message if an error occurs. Add more fine-grained error management here."
            # "Error - Check the error message data and respond accordingly. This message is sent by the \"Error Handler\" VIs at the end of each loop in this application."
            n154 = property on="Property Node" class="Module Admin"(reference=w310) -> ("Accessors:External Launch"=w309:bool)  [unwired: 1 in, 2 out]
            n155 = Variant To Data(error in=w318, type=errorcluster {"status"=FALSE, "code"=0, "source"=""} ("error constant"), Variant=w312) -> (data=w308:errorcluster, error out=w316:errorcluster)
            n156 = local write "error out"(w308) -> ()
            n157 = call "Error Reported.vi"("Error"=w308) -> ()  [unwired: 10 in, 1 out]
            n158 = case shown="False" w309 {
              tunnel: [w323 _] -> w315
              tunnel: w311 -> [w321 _]
              tunnel: w308 -> [w322 _]
              frame False {
                n159 = disable-structure shown="Default" {
                  disable-tunnel: w322 -> [w324 _]
                  frame condition #0 (active) {
                    # "If the module is running standalone, then pop up an error dialog and call the \"Exit\" message."
                    n160 = call <vilib>:"Simple Error Handler.vi"("error in (no error)"=w324) -> ()  [unwired: 4 in, 5 out]
                  }
                  frame condition #1 {
                    # "To prevent the Simple Error Handler VI from being loaded (e.g. when deploying to a Real-Time target), add the Conditional Disable Symbol \"DQMH_Disable_SEH\" to your project and set it to TRUE."
                  }
                }
                n161 = call-poly <vilib>:"Delacor_lib_QMH_Enqueue Message (poly).vi"("Priority Message? (F)"=TRUE, "Message"="Exit", "Message Queue in"=w321) -> ("error out"=w323:errorcluster)  [unwired: 7 in, 1 out]
              }
              frame True {
                # "If the module was launched externally, calling the Error Reported broadcast VI is the only action performed by the \"Error\" message. The module's caller can then process the error appropriately."
              }
            }
            n162 = Merge Errors(w316, w315) -> (w314:errorcluster)
          }
          frame "Exit" {
            w329 = 91  # 91: not all Exit messages will have an argument
            w331 = TRUE  # Stop the VI
            # "Release the message queue reference"
            # "#DQMH_CodeNeeded - Add any required cleanup code here."
            # "Exit - Exit the application."
            n163 = Variant To Data(error in=w339, type=T7 {"Origin"="", "Exit via Stop Module Req?"=FALSE, "Wait for Module to stop?"=FALSE} ("Stop Argument"), Variant=w330) -> (data=w327:T7, error out=w336:errorcluster)
            n164 = call <vilib>:"Clear Errors.vi"("error in (no error)"=w336, "specific error code to clear (0: all)"=w329) -> ("error out"=w338:errorcluster)  [unwired: 4 in, 1 out]
            n165 = control-ref of="This VI"() -> (w326:refnum<vi>)
            n166 = call-dynamic "Delacor_lib_QMH_Release Message Queue.vi"("error in"=w338, "Message Queue"=w333) -> ("error out"=w337:errorcluster)  [unwired: 9 in]
            n167 = call "Handle Exit.vi"("Stop Argument"=w327, "Admin in"=w325, "VI reference"=w326) -> ("error out"=w335:errorcluster)  [unwired: 7 in, 1 out]
            n168 = Merge Errors(w337, w335) -> (w334:errorcluster)
            n169 = call "Error Reported.vi"("Error"=w334) -> ()  [unwired: 10 in, 1 out]
          }
          frame Default {
            # "'Default' case only runs if there is a message that isn't defined in any of the other cases.  Output a programming error."
            n170 = call "Module Name--constant.vi"() -> ("Module Name"=w344:string)  [unwired: 11 in]
            n171 = Format Into String(format string="The invalid message string \"%s\" was received in the Message Handling Loop for module \"%s\".", w345, w344) -> (resulting string=w340:string)  [unwired: 2 in, 1 out]
            n172 = call <vilib>:"Error Cluster From Error Code.vi"("show call chain? (False)"=TRUE, "error message (\"\")"=w340, "error code (0)"=1) -> ("error out"=w347:errorcluster)  [unwired: 6 in]
            n173 = Merge Errors(w348, w347) -> (w349:errorcluster)
          }
        }
        n174 = call-dynamic "Delacor_lib_QMH_Error Handler - Message Handling Loop.vi"("error in"=w152, "Message Queue in"=w151) -> ("dup error in"=w153:errorcluster)  [unwired: 8 in, 1 out]
      }
    }
    frame Error {
      # "Synchronize Caller Events.vi will inform Start Module.vi that the module has launched and will let the code calling Start Module.vi register for broadcasts and would permit the caller receive the broadcast that an error occurred at launch time."
      n175 = call-dynamic "Delacor_lib_QMH_Release Message Queue.vi"("error in"=w357, "Message Queue"=w350) -> ("error out"=w356:errorcluster)  [unwired: 9 in]
      n176 = call "Synchronize Caller Events.vi"("Singleton Module Admin in"=w351) -> ("error out"=w358:errorcluster)  [unwired: 9 in, 1 out]
      n177 = call "Module Name--constant.vi"() -> ("Module Name"=w354:string)  [unwired: 11 in]
      n178 = Format Into String(format string="An error occurred during initialization. %s is no longer running.", w354) -> (resulting string=w352:string)  [unwired: 2 in, 1 out]
      n179 = Merge Errors(w356, w358) -> (w359:errorcluster)
      n180 = call "Error Reported.vi"("Additional Information"=w352, "Error"=w359) -> ()  [unwired: 9 in, 1 out]
    }
  }
  n181 = Merge Errors(w14, w17) -> (w13:errorcluster)
  n182 = call "Close Module.vi"("error in"=w13, "Module Admin in"=w8) -> ("error out"=w15:errorcluster, "External Launch"=w1:bool, "Module Admin out"=w2:refnum<class "Delacor_lib_QMH_Module Admin.lvclass">)  [unwired: 7 in]
  n183 = Unregister For Events(event registration refnum=w7, error in=w15) -> (error out=w12:errorcluster)
  "error out" <- w12
  n184 = case "External Launch?" shown="True" w1 {
    tunnel: w12 -> [_ w360]
    frame False {
    }
    frame True {
      n185 = case shown="No Error" w360 {
        frame No Error {
          n186 = invoke on="Invoke Node" class="VI" method="FP.Close"() -> ()  [unwired: 3 in, 3 out]
        }
        frame Error {
          n187 = disable-structure shown="Default" {
            frame condition #0 (active) {
              n188 = invoke class="VI" method="FP.Open"("Activate"=TRUE ("Activate?")) -> ()  [unwired: 4 in, 5 out]
            }
            frame condition #1 {
              # "Don't show panel on error if running inside a built EXE."
            }
          }
        }
      }
    }
  }
  n189 = local write "Module Admin"(w2) -> ()
